vi "Host_AxisInit.vi"(11 "Motion":refnum<visa-resource-name>) -> (3 "error out":errorcluster)   [LabVIEW 2018]
doc: "Use this template to build a VI to use as a subVI."
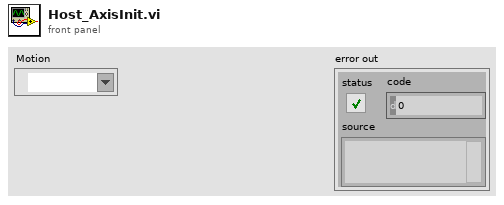
[diagram p1: front panel]
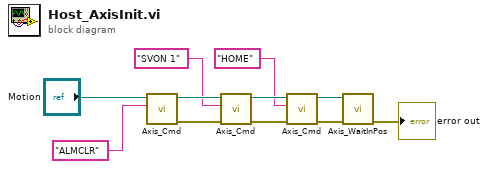
[diagram p0: block diagram]
diagram:
  n1 = call "Axis_Cmd.vi"("Command"="ALMCLR", "VISA Refnum name"="Motion") -> ("error out"=w8:errorcluster, "VISA Refnum name out"=w9:refnum<visa-resource-name>)  [unwired: 7 in, 1 out]
  n2 = call "Axis_Cmd.vi"("error in (no error)"=w8, "Command"="SVON 1", "VISA Refnum name"=w9) -> ("error out"=w5:errorcluster, "VISA Refnum name out"=w6:refnum<visa-resource-name>)  [unwired: 6 in, 1 out]
  n3 = call "Axis_Cmd.vi"("error in (no error)"=w5, "Command"="HOME", "VISA Refnum name"=w6) -> ("error out"=w2:errorcluster, "VISA Refnum name out"=w3:refnum<visa-resource-name>)  [unwired: 6 in, 1 out]
  n4 = call "Axis_WaitInPos.vi"("error in (no error)"=w2, "VISA Refnum name"=w3) -> ("error out"=→"error out":errorcluster)  [unwired: 8 in, 1 out]
